vi "Library Template Name--constant.vi"() -> (3 "Library Template Name":string)   [LabVIEW 2026]
doc: "This constant defines the name of the lvlib template in the main project directory."
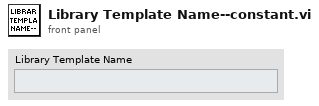
[diagram p1: front panel]
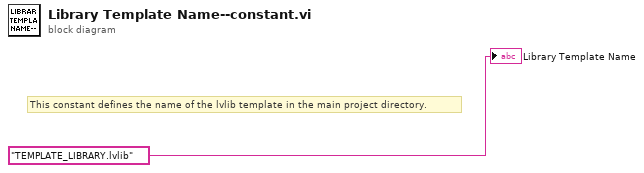
[diagram p0: block diagram]
diagram:
  # "This constant defines the name of the lvlib template in the main project directory."
  "Library Template Name" <- "TEMPLATE_LIBRARY.lvlib"
